vi "VIHelpeks VIs.vi"() -> ()   [LabVIEW 2014]
doc: "::: VI Helpeks :::\nCopyright (c) 2000-2026 Konstantin Shifershteyn. All rights reserved."
uses:
  Project/VI Helpeks/_VIH Project Manager.llb/VIH Project Tree Typedef - Tree Refnum.ctl
  Project/VI Helpeks/_VIH Project Manager.llb/VIH Project Tree Typedef - Tree Item Type.ctl
  <vilib>/Palette API/Palette Menu/Public Type Define/Items.ctl
  <vilib>/Palette API/Palette Menu/Public Type Define/Item.ctl
  Project/VI Helpeks/_VIH HelpGen - Palette.llb/VIH HelpGen Typedef - Palette - Item Type Enum.ctl
  vi.lib/addons/VI Helpeks/VIHelpeksAPI.lvlib
  <vilib>/Palette API/Palette Menu/Palette Menu.lvlib
panel:
  in  "False":bool
  # "VI Collection"
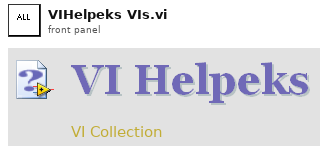
[diagram p1: front panel]
types:
  T1 = typedef "Palette Menu.lvlib/Items.ctl" = T2[]
  T2 = typedef "Palette Menu.lvlib/Item.ctl" = cluster{"item path":path, "library path (.lvlib)":path, "use default lvlib palette":bool, "short name":string, "place VI contents":bool, "hide synchronized item":bool, "reserve spot for synch item":bool, "configure when placing VI contents":bool}
  T3 = enum16{"nop", "Init", "get index", "get symbols"}
  T4 = typedef "VIH HelpGen Typedef - Palette - Item Type Enum.ctl" = enum32{"<Invalid>", "<unknown>", "VI", "Menu", "LV Func", "Express VI", "Poly VI", "CTL", "HTML"}
  T5 = typedef "VIH Project Tree Typedef - Tree Item Type.ctl" = enum32{"<Invalid>", "Project", "Proj Files", "Proj Rules", "File Group", "Rule Group", "Any File", "LV Func", ".mnu", ".mnu (dyn)", ".vi", ".vi (dyn)", ".vit", ".vit (dyn)", ".ctl", ".ctl (dyn)", ".ctt", ".ctt (dyn)", "polyVI", "polyVI (dyn)", "expVI", "expVI (dyn)", "HTML", "PolyVI Inst"}
  T6 = typedef "VIH Project Tree Typedef - Tree Refnum.ctl" = refnum<vi>
  T7 = cluster{"Source File Name":string, "Source File Path":path, "HTML File Path":path, "CHM Local Path":string, "CHM Keyword":string}[]
  T8 = cluster{"Help Path":path, "Help Tag":string, "Abs Help Path":path}[]
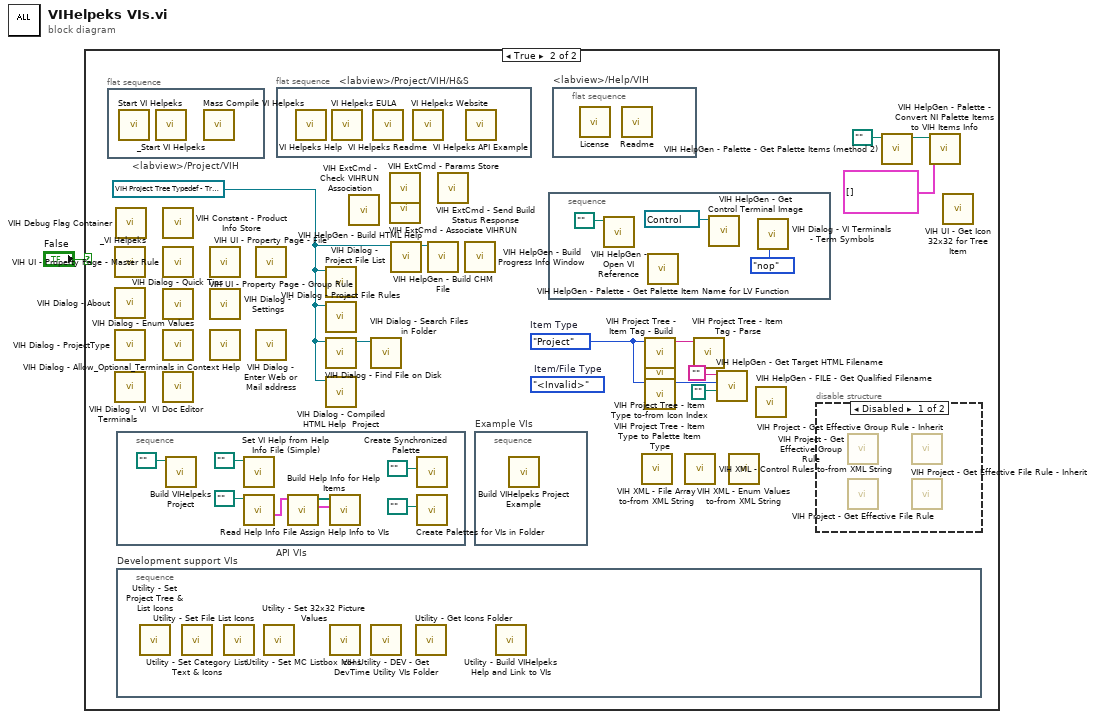
[diagram p0: block diagram]
diagram:
  n1 = case shown="True" "False" {
    frame False {
    }
    frame True {
      (unwired) VIH_HelpGen_Typedef_-_Palette_-_Item_Type_Enum."<Invalid>"  # Item/File Type
      w11 = VIH_Project_Tree_Typedef_-_Tree_Item_Type."Project"  # Item Type
      w9 = T6 refnum ("Project Tree")
      n2 = flat-sequence "<labview>/Project/VIH" {
        frame #0 {
          n3 = call "Start VI Helpeks.vi"() -> ()  [unwired: 12 in]
          n4 = call "_Start VI Helpeks.vi"() -> ()  [unwired: 12 in]
          n5 = call "Mass Compile VI Helpeks.vi"() -> ()  [unwired: 1 in]
        }
      }
      n6 = call "_VI Helpeks.vi"() -> ()  [unwired: 12 in]
      n7 = call "VIH Dialog - About.vi"() -> ()  [unwired: 11 in, 1 out]
      n8 = call "VIH Dialog - ProjectType.vi"() -> ()  [unwired: 10 in, 2 out]
      n9 = call "VIH Dialog - VI Terminals.vi"() -> ()  [unwired: 8 in, 4 out]
      n10 = call "VIH Debug Flag Container.vi"() -> ()  [unwired: 11 in, 1 out]
      n11 = stacked-sequence "API VIs" {
        frame #0 {
          n12 = call "Build VIHelpeks Project.vi"("VIHelpeks Project File"=path "" ("VIHelpeks Project file")) -> ()  [unwired: 7 in, 4 out]
          n13 = call "Set VI Help from Help Info File (Simple).vi"("Help Info File"=path "") -> ()  [unwired: 7 in, 4 out]
          n14 = call "Read Help Info File.vi"("Help Info File"=path "") -> ("Help Items"=w16:T7)  [unwired: 7 in, 3 out]
          n15 = call "Build Help Info for Help Items.vi"("Help Items"=w16) -> ("Source Files Help Info"=w13:T8, "Source File Paths"=w14:path[])  [unwired: 8 in, 1 out]
          n16 = call "Assign Help Info to VIs.vi"("Source Files Help Info"=w13, "Source File Paths"=w14) -> ()  [unwired: 7 in, 3 out]
          n17 = call "Create Synchronized Palette.vi"("Folder Path"=path "") -> ()  [unwired: 8 in, 3 out]
          n18 = call "Create Palettes for VIs in Folder.vi"("Folder or LLB Path"=path "" ("Folder or LLB")) -> ()  [unwired: 8 in, 3 out]
        }
      }
      n19 = stacked-sequence "Development support VIs" {
        frame #0 {
          n20 = call "Utility - Set Project Tree & List Icons.vi"() -> ()  [unwired: 10 in, 2 out]
          n21 = call "Utility - Set Category List Text & Icons.vi"() -> ()  [unwired: 11 in, 1 out]
          n22 = call "Utility - Set File List Icons.vi"() -> ()  [unwired: 11 in, 1 out]
          n23 = call "Utility - Set 32x32 Picture Values.vi"() -> ()  [unwired: 11 in, 1 out]
          n24 = call "Utility - Set MC Listbox Icons.vi"() -> ()  [unwired: 11 in, 1 out]
          n25 = call "VIH Utility - DEV - Get DevTime Utility VIs Folder.vi"() -> ()  [unwired: 9 in, 3 out]
          n26 = call "Utility - Get Icons Folder.vi"() -> ()  [unwired: 10 in, 2 out]
          n27 = call "Utility - Build VIHelpeks Help and Link to VIs.vi"() -> ()  [unwired: 12 in]
        }
      }
      n28 = call "VIH Constant - Product Info Store.vi"() -> ()  [unwired: 1 out]
      n29 = call "VIH UI - Property Page - Master Rule.vi"() -> ()  [unwired: 12 in]
      n30 = call "VIH Dialog - Quick Tips.vi"() -> ()  [unwired: 10 in, 2 out]
      n31 = call "VIH Dialog - Enum Values.vi"() -> ()  [unwired: 10 in, 2 out]
      n32 = call "VI Doc Editor.vi"() -> ()  [unwired: 10 in, 2 out]
      n33 = call "VIH UI - Property Page - Group Rule.vi"() -> ()  [unwired: 12 in]
      n34 = call "VIH Dialog - Settings.vi"() -> ()  [unwired: 11 in, 1 out]
      n35 = call "VIH Dialog - Allow_Optional_Terminals in Context Help.vi"() -> ()  [unwired: 11 in, 1 out]
      n36 = call "VIH UI - Property Page - File.vi"() -> ()  [unwired: 12 in]
      n37 = call "VIH Dialog - Enter Web or Mail address.vi"() -> ()  [unwired: 9 in, 3 out]
      n38 = flat-sequence "<labview>/Project/VIH/H&S" {
        frame #0 {
          n39 = call "VI Helpeks Help.vi"() -> ()  [unwired: 12 in]
          n40 = call "VI Helpeks EULA.vi"() -> ()  [unwired: 12 in]
          n41 = call "VI Helpeks Readme.vi"() -> ()  [unwired: 12 in]
          n42 = call "VI Helpeks Website.vi"() -> ()  [unwired: 12 in]
          n43 = call "VI Helpeks API Example.vi"() -> ()  [unwired: 12 in]
        }
      }
      n44 = call "VIH Dialog - Project File List.vi"("Project Tree"=w9) -> ()  [unwired: 8 in, 3 out]
      n45 = call "VIH Dialog - Project File Rules.vi"("Project Tree"=w9) -> ()  [unwired: 9 in, 2 out]
      n46 = call "VIH Dialog - Find File on Disk.vi"("Project Tree"=w9) -> ("dup Project Tree"=w10:T6)  [unwired: 7 in, 3 out]
      n47 = call "VIH Dialog - Compiled HTML Help  Project.vi"("Project Tree"=w9) -> ()  [unwired: 11 in]
      n48 = call "VIH ExtCmd - Check VIHRUN Association.vi"() -> ()  [unwired: 7 in, 5 out]
      n49 = call "VIH Dialog - Search Files in Folder.vi"("Project Tree"=w10) -> ()  [unwired: 7 in, 4 out]
      n50 = call "VIH ExtCmd - Params Store.vi"() -> ()  [unwired: 10 in, 2 out]
      n51 = call "VIH ExtCmd - Associate VIHRUN.vi"() -> ()  [unwired: 11 in, 1 out]
      n52 = call "VIH HelpGen - Build HTML Help.vi"("Project Tree"=w9) -> ("dup Project Tree"=w8:T6)  [unwired: 9 in, 1 out]
      n53 = call "VIH HelpGen - Build CHM File.vi"("Project Tree"=w8) -> ()  [unwired: 7 in, 4 out]
      n54 = call "VIH ExtCmd - Send Build Status Response.vi"() -> ()  [unwired: 11 in, 1 out]
      n55 = call "VIH HelpGen - Build Progress Info Window.vi"() -> ()  [unwired: 11 in, 1 out]
      n56 = stacked-sequence "Example VIs" {
        frame #0 {
          n57 = call "Build VIHelpeks Project Example.vi"() -> ()  [unwired: 8 in, 4 out]
        }
      }
      n58 = stacked-sequence {
        frame #0 {
          n59 = call "VIH HelpGen - Open VI Reference.vi"("VI Path"=path "") -> ()  [unwired: 7 in, 4 out]
          n60 = call "VIH HelpGen - Palette - Get Palette Item Name for LV Function.vi"() -> ()  [unwired: 9 in, 3 out]
          n61 = call "VIH HelpGen - Get Control Terminal Image.vi"("Ctl Refnum"=refnum<vi> refnum) -> ()  [unwired: 6 in, 5 out]
          n62 = call "VIH Dialog - VI Terminals - Term Symbols.vi"("cmd (nop)"=T3."nop") -> ()  [unwired: 7 in, 4 out]
        }
      }
      n63 = flat-sequence "<labview>/Help/VIH" {
        frame #0 {
          n64 = call "License.vi"() -> ()  [unwired: 12 in]
          n65 = call "Readme.vi"() -> ()  [unwired: 12 in]
        }
      }
      n66 = call "VIH XML - File Array to-from XML String.vi"() -> ()  [unwired: 8 in, 4 out]
      n67 = call "VIH Project Tree - Item Tag - Build.vi"("Item Type"=w11) -> ("Tree Item Tag"=w12:string)  [unwired: 9 in, 1 out]
      n68 = call "VIH Project Tree - Item Type to-from Icon Index.vi"() -> ()  [unwired: 11 in, 1 out]
      n69 = call "VIH Project Tree - Item Type to Palette Item Type.vi"("Tree Item Type"=w11) -> ("Item/File Type"=w7:T4)  [unwired: 9 in, 1 out]
      n70 = call "VIH XML - Control Rules to-from XML String.vi"() -> ()  [unwired: 8 in, 4 out]
      n71 = call "VIH Project Tree - Item Tag - Parse.vi"("Tree Item Tag"=w12) -> ()  [unwired: 8 in, 3 out]
      n72 = call "VIH HelpGen - Get Target HTML Filename.vi"("Item File Path"=path "", "Item Type"=w7, "HTML Filename in"="") -> ()  [unwired: 7 in, 2 out]
      n73 = call "VIH XML - Enum Values to-from XML String.vi"() -> ()  [unwired: 8 in, 4 out]
      n74 = call "VIH HelpGen - FILE - Get Qualified Filename.vi"() -> ()  [unwired: 10 in, 2 out]
      n75 = disable-structure shown="Disabled" {
        frame Disabled {
          n76 = call "VIH Project - Get Effective Group Rule.vi"() -> ()  [unwired: 9 in, 3 out]
          n77 = call "VIH Project - Get Effective File Rule.vi"() -> ()  [unwired: 8 in, 4 out]
          n78 = call "VIH Project - Get Effective Group Rule - Inherit.vi"() -> ()  [unwired: 11 in, 1 out]
          n79 = call "VIH Project - Get Effective File Rule - Inherit.vi"() -> ()  [unwired: 11 in, 1 out]
        }
        frame Enabled {
        }
      }
      n80 = call "VIH HelpGen - Palette - Get Palette Items (method 2).vi"("Palette Path"=path "") -> ("dup Palette Path"=w3:path)  [unwired: 8 in, 2 out]
      n81 = call "VIH HelpGen - Palette - Convert NI Palette Items to VIH Items Info.vi"("Palette Items"=T1 [], "Palette Path"=w3) -> ()  [unwired: 7 in, 3 out]
      n82 = call "VIH UI - Get Icon 32x32 for Tree Item.vi"() -> ()  [unwired: 10 in, 2 out]
    }
  }
